vi "Restore Data.vi"(8 "error in":errorcluster, 11 "Module ID":i32=-1) -> (0 "error out":errorcluster)   [LabVIEW 2020, in "Data Viewer.lvlib"]
doc: "_____\nCreated using DQMH Event Scripter 7.0.1.1316."
uses:
  Data Viewer.lvlib
  Restore Data Argument--cluster.ctl
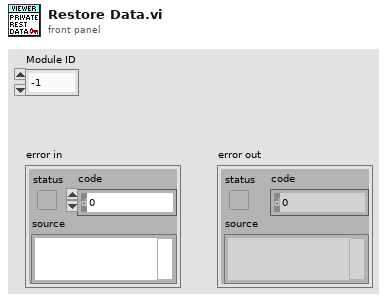
[diagram p1: front panel]
types:
  T1 = typedef "Data Viewer.lvlib/Restore Data Argument--cluster.ctl" = cluster{"Module ID":i32, "布尔":bool}
  T2 = typedef "Data Viewer.lvlib/Request Events--cluster.ctl" = cluster{"Stop Module":refnum<user-event>, "Show Panel":refnum<user-event>, "Hide Panel":refnum<user-event>, "Show Diagram":refnum<user-event>, "Get Module Execution Status":refnum<user-event>, "Private":cluster{"Window Resize":refnum<user-event>, "Open File":refnum<user-event>, "Draw Plot":refnum<user-event>, "Set YScale":refnum<user-event>, "Update Curve Color":refnum<user-event>, "Show Value":refnum<user-event>, "Menu Action":refnum<user-event>, "Update Filter Arguments":refnum<user-event>, "Filte Data":refnum<user-event>, "Restore Data":refnum<user-event>, "Cut Half Data":refnum<user-event>, "Select Point":refnum<user-event>, "Open Linear Measurement":refnum<user-event>, "Linear Measurement Close":refnum<user-event>}, "Scale List Menu Action":refnum<user-event>, "Private.Update Scale List":refnum<user-event>, "Private.Initialize Plot List":refnum<user-event>, "Private.Load Plot":refnum<user-event>, "Private.Unload Plot":refnum<user-event>, "Show Hide Scale":refnum<user-event>, "Private.Add Default Scale":refnum<user-event>, "Private.Update Plot List":refnum<user-event>, "Private.Add Virtual Cruve":refnum<user-event>, "Private.Edit Curve":refnum<user-event>}
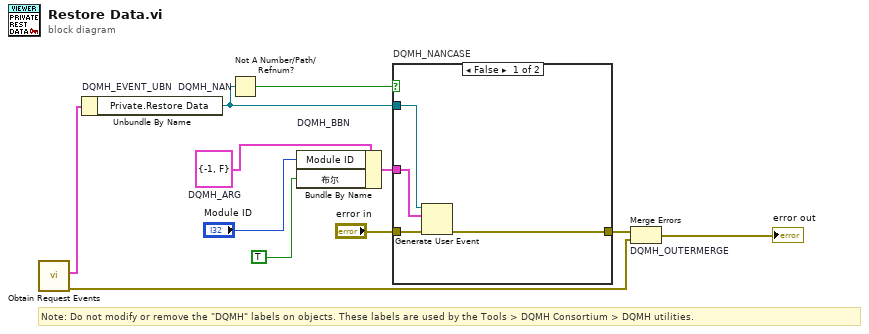
[diagram p0: block diagram]
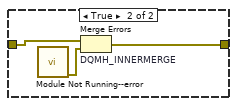
[diagram p2: hidden frame]
diagram:
  w5 = T1 {"Module ID"=-1, "布尔"=FALSE}  # DQMH_ARG
  # "Note: Do not modify or remove the \"DQMH\" labels on objects. These labels are used by the Tools > DQMH Consortium > DQMH utilities."
  n1 = call "Obtain Request Events.vi"() -> ("error out"=w2:errorcluster, "Data Viewer Request Events"=w1:T2)  [unwired: 10 in]
  n2 = Unbundle By Name "DQMH_EVENT_UBN"(w1) -> ("Private.Restore Data"=w7:refnum<user-event>)
  n3 = Not A Number/Path/Refnum? "DQMH_NAN"(number/path/refnum=w7) -> (NaN/Path/Refnum?=w8:bool)
  n4 = Bundle By Name "DQMH_BBN"(cluster=w5, "Module ID"="Module ID", "布尔"=TRUE) -> (w9:T1)
  n5 = case "DQMH_NANCASE" shown="False" w8 {
    tunnel: "error in" -> [w15 w18]
    tunnel: [w14 w17] -> w6
    tunnel: w7 -> [w13 _]
    tunnel: w9 -> [w12 _]
    frame False {
      n6 = Generate User Event(user event=w13, event data cluster=w12, error in=w15) -> (error out=w14:errorcluster)  [unwired: 1 in, 1 out]
    }
    frame True {
      n7 = call "Module Not Running--error.vi"() -> ("error out"=w16:errorcluster)  [unwired: 11 in]
      n8 = Merge Errors "DQMH_INNERMERGE"(w18, w16) -> (w17:errorcluster)
    }
  }
  n9 = Merge Errors "DQMH_OUTERMERGE"(w6, w2) -> (→"error out":errorcluster)
